vi "Read ExpressionWithTags.vi"(8 "error in (no error)":errorcluster, 11 "muExpr in":refnum<class "Tag Expr.lvclass">) -> (0 "error out":errorcluster, 2 "Expression":string, 3 "muExpr out":refnum<class "Tag Expr.lvclass">)   [LabVIEW 2020, in "Tag Expr.lvclass"]
doc: "Returns the expression as it was passed to Construct, with ${TAG_NAME} references. It does not return the placeholder version that is passed to muParser."
uses:
  Tag Expr.lvclass
  Tag Expr.lvclass/Tag Expr.ctl
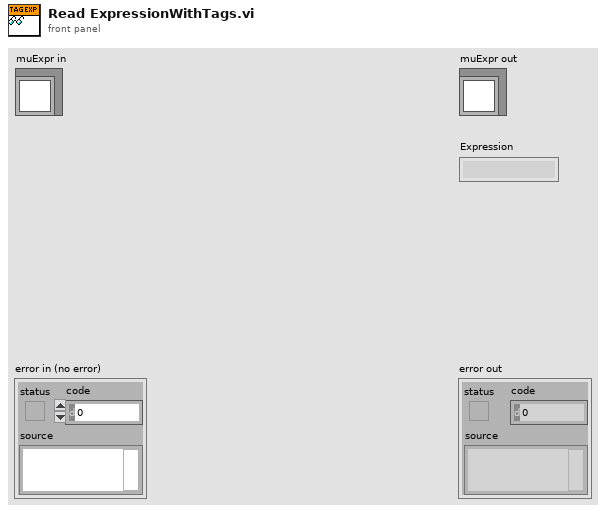
[diagram p1: front panel]
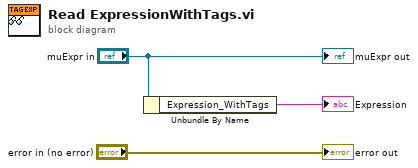
[diagram p0: block diagram]
diagram:
  n1 = Unbundle By Name("muExpr in") -> ("Expression_WithTags"=→"Expression":string)
  "error out" <- "error in (no error)"
  "muExpr out" <- "muExpr in"
